vi "pi_golden3.vi"() -> ()   [LabVIEW 2020]
panel:
  out "PI1":dbl
  out "PI0":dbl
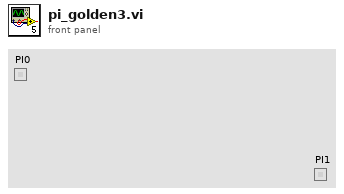
[diagram p1: front panel]
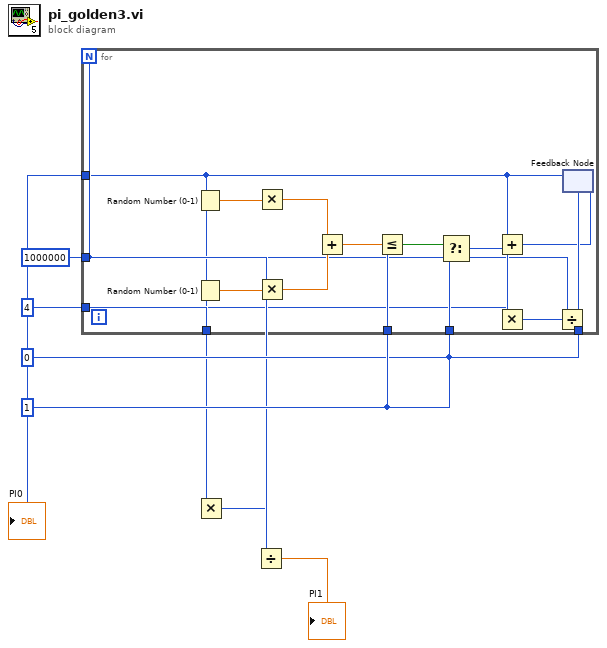
[diagram p0: block diagram]
diagram:
  w8 = 1 ("OneConst")
  w7 = 0 ("ZeroConst")
  w6 = 4 ("FourConst")
  w5 = 1000000 ("NConst")
  n1 = for "Loop1" {
    N: w5 -> [_]
    tunnel: w8 -> [w24]
    tunnel: w7 -> [w23]
    tunnel: w8 -> [w22]
    tunnel: w7 -> [w21]
    tunnel: w6 -> [w12]
    tunnel: w5 -> [w10]
    tunnel: [w9] -> w4
    tunnel: [w9] -> w3
    n2 = Random Number (0-1) ("RN1")() -> (number: 0 to 1=w20:dbl)
    n3 = Random Number (0-1) ("RN2")() -> (number: 0 to 1=w19:dbl)
    n4 = Multiply ("SQX")(x=w20, y=w20) -> (x*y=w18:dbl)
    n5 = Multiply ("SQY")(x=w19, y=w19) -> (x*y=w17:dbl)
    n6 = Add ("R2")(x=w18, y=w17) -> (x+y=w16:dbl)
    n7 = Less Or Equal? ("LE1")(x=w16, y=w24) -> (x <= y?=w15:bool)
    n8 = Select ("SEL1")(t=w22, s=w15, f=w23) -> (s? t:f=w14:i32)
    n9 = feedback #1 ("FN1")(w21) -> (w9:i32)
    n10 = Add ("ACC")(x=w9, y=w14) -> (x+y=w13:i32)
    n11 = Multiply ("P")(x=w12, y=w13) -> (x*y=w11:i32)
    n12 = Divide ("DIV")(x=w11, y=w10) -> ()  [unwired: 1 out]
    n13 = feedback-in #1(w13) -> ()
  }
  "PI0" <- w4
  n14 = Multiply ("MUL4")(x=w3, y=w6) -> (x*y=w2:i32)
  n15 = Divide ("DIV2")(x=w2, y=w5) -> (x/y=→"PI1":dbl)
